vi "update channel metadata.vi"(6 "clear unit":bool, 8 "Unit":string, 9 "Description":string, 10 "Channel":refnum<class "Channel.lvclass">, 11 "connection":refnum<class "Nominal Client.lvclass">) -> (0 "error out":errorcluster)   [LabVIEW 2020, in "nominal core steps.lvlib"]
doc: "Update channel's description and unit. Clear unit takes precedence over any value set in the unit field."
uses:
  nominal core steps.lvlib
  <vilib>/Nominal/Nominal IO Client/submodules/nominal-streaming-labview-ffi/lv_src/Channel/Channel.lvclass
  <vilib>/Nominal/Nominal IO Client/lv_src/Nominal Client/Nominal Client.lvclass
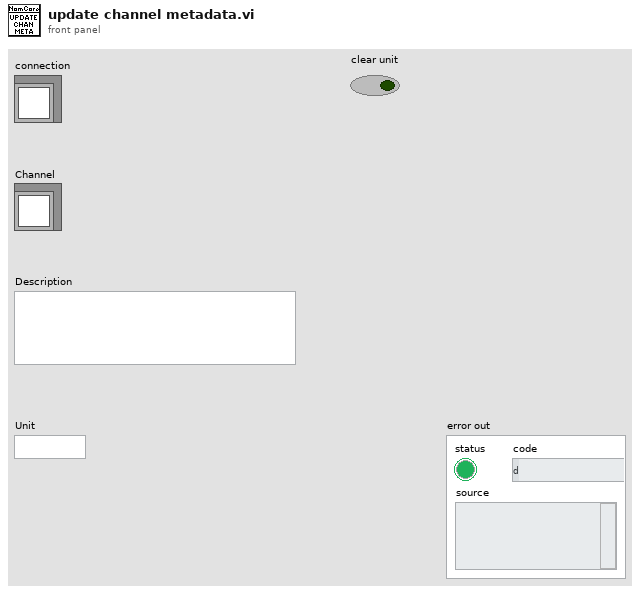
[diagram p1: front panel]
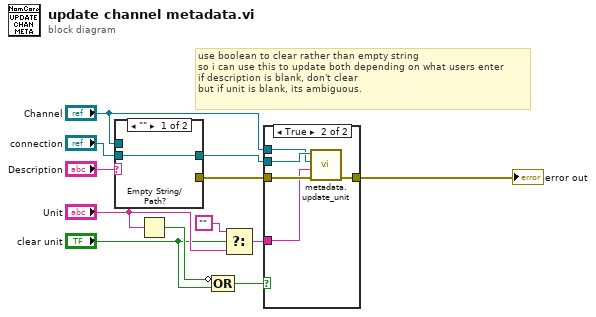
[diagram p0: block diagram]
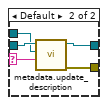
[diagram p3: hidden frame]
diagram:
  # "use boolean to clear rather than empty string\nso i can use this to update both depending on what users enter\nif description is blank, don't clear\nbut if unit is blank, its ambiguous."
  n1 = case shown="\"\"" "Description" {
    selector: "Description" -> [_ w14]
    tunnel: "connection" -> [w13 w18]
    tunnel: [w13 w17] -> w11
    tunnel: [_ w16] -> w10
    tunnel: "Channel" -> [_ w15]
    frame "" {
    }
    frame Default {
      n2 = call <vilib>:"metadata.update_description.vi"("Description"=w14, "Channel"=w15, "Nominal Client in"=w18) -> ("error out"=w16:errorcluster, "Nominal Client out"=w17:refnum<class "Nominal Client.lvclass">)  [unwired: 6 in, 1 out]
    }
  }
  n3 = Empty String/Path?(string/path="Unit") -> (empty?=w4:bool)
  n4 = Compound Arithmetic op=OR(invert w4, "clear unit") -> (w2:bool)
  n5 = Select(t="", s="clear unit", f="Unit") -> (s? t:f=w1:string)
  n6 = case shown="True" w2 {
    tunnel: w11 -> [_ w24]
    tunnel: w10 -> [w19 w23]
    tunnel: [w19 w22] -> w9
    tunnel: "Channel" -> [_ w21]
    tunnel: w1 -> [_ w20]
    frame False {
    }
    frame True {
      n7 = call <vilib>:"metadata.update_unit.vi"("error in"=w23, "Unit (empty to clear)"=w20, "Channel"=w21, "Nominal Client in"=w24) -> ("error out"=w22:errorcluster)  [unwired: 5 in, 2 out]
    }
  }
  "error out" <- w9
